vi "Create Test Configuration.vi"() -> (0 "error out":errorcluster, 1 "channel names":string[](array[string]), 2 "Lines":T1[](array[typedef]), 3 "Module Configuration":refnum<class "Shared Memory configuration.lvclass">, 4 "Channels":refnum<class "TBM channel.lvclass">[](array[class]), 5 "instance identifier":string, 6 "Channels?":bool, 7 "instance identifier?":bool, 8 "Lines?":bool)   [LabVIEW 2014, in "Shared Memory tests.lvlib"]
doc: "This VI creates a standard test configuration for other unit tests. It currently creates and adds one line with every datatype to the module configuration."
uses:
  Shared Memory tests.lvlib
  module/configuration/Shared Memory configuration.lvclass
  module/configuration/Line.ctl
  <vilib>/NI/Tag Bus Module Framework/channel/TBM channel.lvclass
  module/configuration/Shared Memory configuration.lvclass/Shared Memory configuration.ctl
  module/configuration/Write Input File String.vi
  module/configuration/Write Output File String.vi
  module/configuration/Write sync struct name.vi
  <vilib>/NI/Configuration Framework/serializable configuration/NISE_CEF_serializable configuration.lvclass
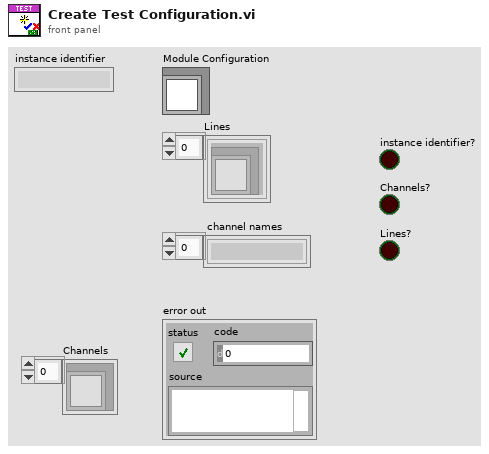
[diagram p1: front panel]
types:
  T1 = typedef "Shared Memory configuration.lvclass/Line.ctl" = cluster{"channel":refnum<class "TBM channel.lvclass">}
  T2 = typedef "tag bus.lvlib/tag descriptor.lvclass/Data Type.ctl" = enum16{"Double", "Single", "I64", "I32", "I16", "I8", "U64", "U32", "U16", "U8", "Boolean", "String", "Array of Double", "Array of Single", "Array of I64", "Array of I32", "Array of I16", "Array of I8", "Array of U64", "Array of U32", "Array of U16", "Array of U8", "Array of Boolean", "Array of String"}
  T3 = typedef "TBM channel.lvclass/channel classification.ctl" = enum16{"input data", "output data", "processing parameter", "processing result"}
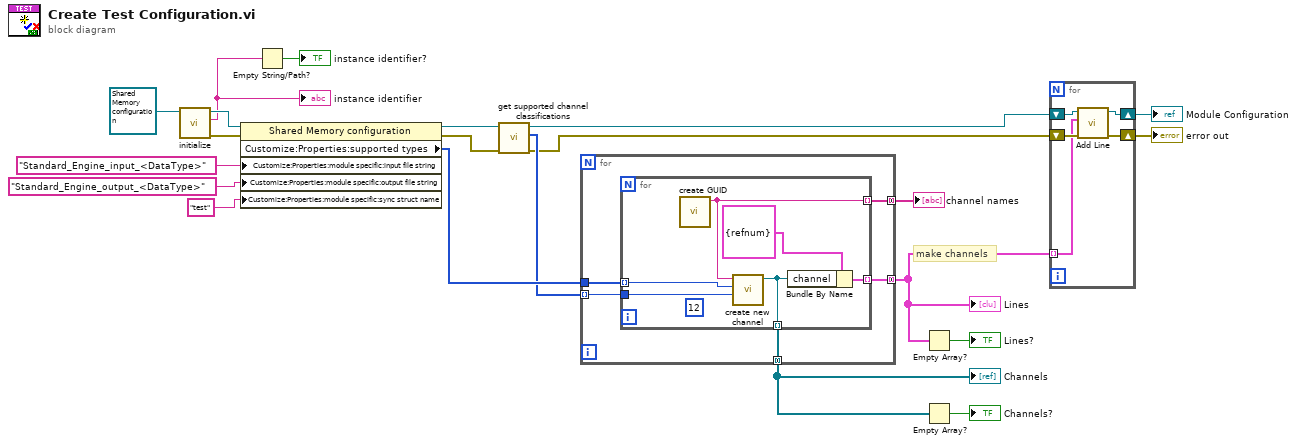
[diagram p0: block diagram]
diagram:
  # "make channels"
  n1 = call <vilib>:"initialize.vi"("configuration in"=refnum<class "Shared Memory configuration.lvclass"> refnum ("tag bus configurable plugin module configuration")) -> ("error out"=w20:errorcluster, "identifier"=w6:string, "configuration out"=w18:refnum<class "Shared Memory configuration.lvclass">)  [unwired: 8 in]
  "instance identifier" <- w6
  n2 = property class="Shared Memory configuration"(reference=w18, error in=w20, "Customize:Properties:module specific:input file string"="Standard_Engine_input_<DataType>", "Customize:Properties:module specific:output file string"="Standard_Engine_output_<DataType>", "Customize:Properties:module specific:sync struct name"="test" ("sync struct name")) -> (reference out=w12:refnum<class "Shared Memory configuration.lvclass">, error out=w9:errorcluster, "Customize:Properties:supported types"=w16:T2[])
  n3 = Empty String/Path?(string/path=w6) -> (empty?=→"instance identifier?":bool)
  n4 = call-dynamic "get supported channel classifications.vi"("error in"=w9, "module configuration in"=w12) -> ("error out"=w8:errorcluster, "supported classes"=w10:T3[], "module configuration out"=w11:refnum<class "Shared Memory configuration.lvclass">)  [unwired: 7 in]
  n5 = for {
    tunnel: w10 -> [w26] mode=indexing
    tunnel: [w24] -> w2 mode=concatenating
    tunnel: w16 -> [w25]
    tunnel: [w23] -> w19 mode=concatenating
    tunnel: [w22] -> w4 mode=concatenating
    n6 = for {
      tunnel: w26 -> [w32]
      tunnel: [w28] -> w24 mode=indexing
      tunnel: w25 -> [w31] mode=indexing
      tunnel: [w30] -> w23 mode=indexing
      tunnel: [w27] -> w22 mode=indexing
      (unwired) 12
      n7 = call <vilib>:"create GUID.vi"() -> ("uuid"=w30:string)  [unwired: 10 in, 1 out]
      n8 = call <vilib>:"create new channel.vi"("channel classification"=w32, "data type"=w31, "channel name"=w30) -> ("channel"=w27:refnum<class "TBM channel.lvclass">)  [unwired: 8 in]
      n9 = Bundle By Name(cluster=T1 {"channel"=refnum} ("Line"), "channel"=w27) -> (w28:T1)
    }
  }
  "channel names" <- w19
  "Lines" <- w2
  "Channels" <- w4
  n10 = Empty Array?(array=w2) -> (empty?=→"Lines?":bool)
  n11 = Empty Array?(array=w4) -> (empty?=→"Channels?":bool)
  n12 = for {
    tunnel: w2 -> [w33] mode=indexing
    shift-right: [w36] -> w17
    shift-left: w11 -> [w37]
    shift-right: [w34] -> w21
    shift-left: w8 -> [w35]
    n13 = call "Add Line.vi"("error in"=w35, "Line"=w33, "Shared Memory configuration in"=w37) -> ("error out"=w34:errorcluster, "Shared Memory configuration out"=w36:refnum<class "Shared Memory configuration.lvclass">)  [unwired: 6 in, 1 out]
  }
  "error out" <- w21
  "Module Configuration" <- w17
